vi "Add ToastActivation Info.vi"(8 "error in (no error)":errorcluster, 9 "activationType":i32(ring) items=["Foreground", "Background", "Protocol"], 10 "launchArgs":string, 11 "reference":refnum<k24>) -> (0 "error out":errorcluster, 3 "reference out":refnum<k24>)   [LabVIEW 2026, in "ToastNotification.lvlib" / "Toast Native.lvlib"]
doc: "Sets the toast body launch arguments and activation type on a borrowed Microsoft.Toolkit.Uwp.Notifications.ToastContentBuilder through AddToastActivationInfo(String launchArgs, ToastActivationType activationType). This replaces the body launch string; it is not an append operation and does not configure individual button arguments. Foreground/Background use application-defined arguments, while Protocol uses a URI handled by Windows. reference out aliases the input builder: no builder handle is acquired or closed here. Displayed text, activation arguments and submitted User Inputs are separate data."
uses:
  Toast Native.lvlib
  C:/Users/loicw/Documents/LabVIEW/ToastNotifications/Sources/bins/Microsoft.Toolkit.Uwp.Notifications.dll
  bins/Microsoft.Toolkit.Uwp.Notifications.dll
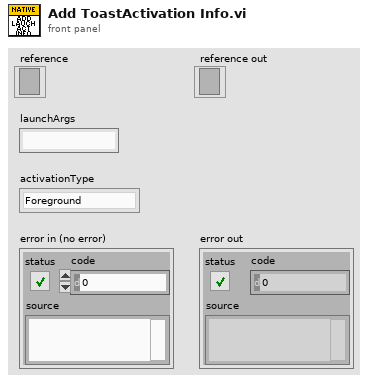
[diagram p1: front panel]
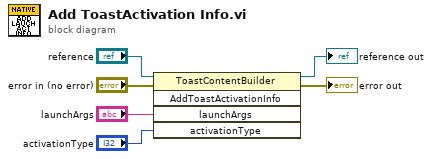
[diagram p0: block diagram]
diagram:
  n1 = invoke class="ToastContentBuilder" method="AddToastActivationInfo"(reference="reference", error in="error in (no error)", "launchArgs"="launchArgs", "activationType"="activationType") -> (reference out=→"reference out":refnum<k24>, error out=→"error out":errorcluster)  [unwired: 1 in, 3 out]
